vi "Test Task Rows.vi"(8 "error in":errorcluster, 10 "Work Folder":path, 11 "Test Data Folder":path) -> (0 "error out":errorcluster, 2 "Report":string, 3 "Passed":bool)   [LabVIEW 2026]
doc: "Tests Project Task Rows.vi and Apply Task Rows.vi on a copy of the schema-v2 sample data. Every check after a write reads the data back from disk with a fresh Initialize Stores.vi (Test - Read Task Rows.vi). The Meetings case and the unknown-ID case each run on their own copy. Checks: Client Website lists Design, Development and Testing in Sort Order with Testing inactive; Testing set active and Meetings (TimeTracker) set inactive survive re-reading; a new name (given with spaces, then repeated with Active FALSE) is added once and stays active; empty and blank names are ignored; tasks not in the rows keep their IDs and Active; an unknown Project ID gives error 5102 and leaves Tasks.ini as the sample it was copied from.\n\nInputs: Test Data Folder; Work Folder; error in. Outputs: Passed; Report; error out.\n\nGenerated by: Claude"
uses:
  UI Support/Task Edit Row.ctl
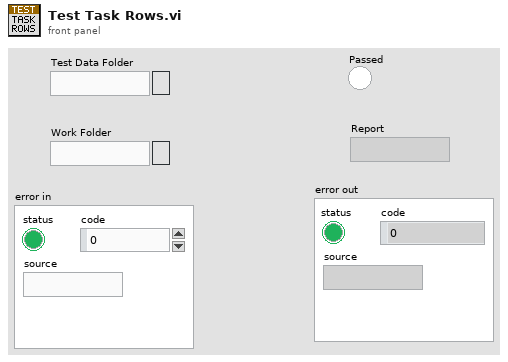
[diagram p1: front panel]
types:
  T1 = typedef "Task Edit Row.ctl" = cluster{"Task Name":string, "Active":bool}
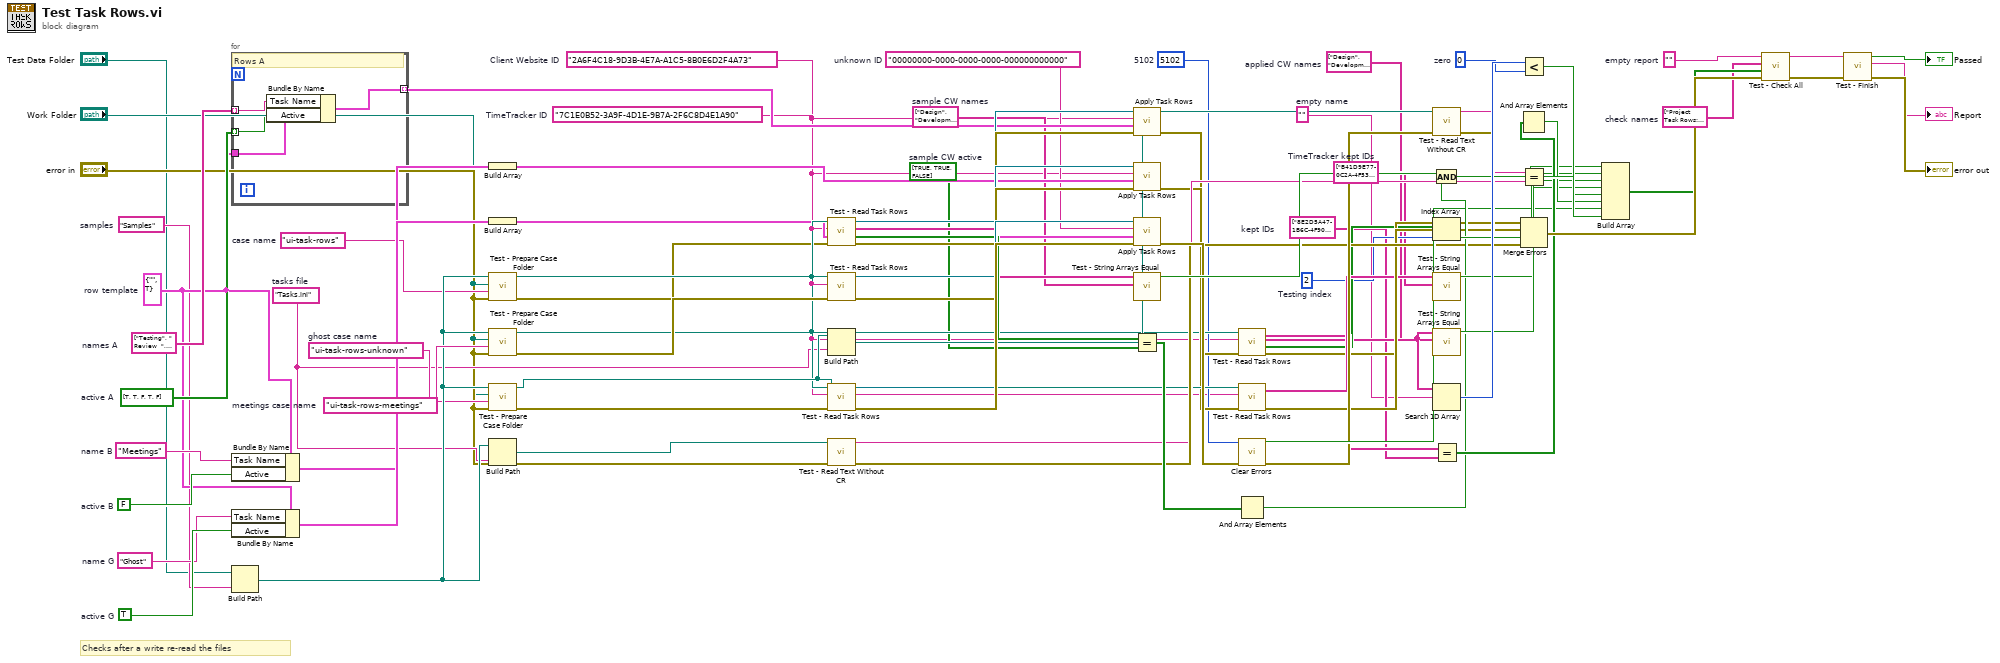
[diagram p0: block diagram]
diagram:
  w55 = "ui-task-rows-meetings"  # meetings case name
  w32 = "ui-task-rows-unknown"  # ghost case name
  w31 = 2  # Testing index
  w30 = string[] ["8E2D5A47-1B6C-4F90-8D3A-7C4B0E9F2A16", "14B9E6D3-A07C-4D52-9F18-3E6A5C2B8D70"]  # kept IDs
  w29 = string[] ["B41D9E77-0C2A-4F53-8E16-5A9D3C7B2E04", "5D8A2C90-7E14-4A6B-B3F9-0C6E1A4D7B25"]  # TimeTracker kept IDs
  w27 = string[] ["Project Task Rows: Client Website gives Design/Development/Testing in Sort Order with Testing inactive", "Apply Task Rows: Testing set active survives re-reading", "Apply Task Rows: Meetings set inactive survives re-reading", "Apply Task Rows: a new name is added once and a repeat in the rows is skipped", "Apply Task Rows: empty and blank names are ignored", "Apply Task Rows: tasks not in the rows keep their IDs and Active", "Apply Task Rows: unknown Project ID gives error 5102", "Apply Task Rows: unknown Project ID leaves Tasks.ini unchanged"]  # check names
  w26 = 5102  # 5102
  w25 = 0  # zero
  w24 = ""  # empty name
  w23 = string[] ["Design", "Development", "Testing", "Review"]  # applied CW names
  w22 = bool[] [TRUE, TRUE, FALSE]  # sample CW active
  w21 = string[] ["Design", "Development", "Testing"]  # sample CW names
  w20 = TRUE  # active G
  w19 = "Ghost"  # name G
  w18 = FALSE  # active B
  w17 = "Meetings"  # name B
  w16 = bool[] [TRUE, TRUE, FALSE, TRUE, FALSE]  # active A
  w15 = string[] ["Testing", "  Review  ", "Review", "", "   "]  # names A
  w14 = T1 {"Task Name"="", "Active"=TRUE}  # row template
  w13 = "00000000-0000-0000-0000-000000000000"  # unknown ID
  w12 = "7C1E0B52-3A9F-4D1E-9B7A-2F6C8D4E1A90"  # TimeTracker ID
  w11 = "2A6F4C18-9D3B-4E7A-A1C5-8B0E6D2F4A73"  # Client Website ID
  w10 = ""  # empty report
  w9 = "Tasks.ini"  # tasks file
  w8 = "ui-task-rows"  # case name
  w7 = "Samples"  # samples
  # "Checks after a write re-read the files"
  n1 = for {
    tunnel: w15 -> [w85] mode=indexing
    tunnel: w16 -> [w86] mode=indexing
    tunnel: w14 -> [w87]
    tunnel: [w88] -> w28 mode=indexing
    # "Rows A"
    n2 = Bundle By Name(cluster=w87, "Task Name"=w85, "Active"=w86) -> (w88:T1)
  }
  n3 = Bundle By Name(cluster=w14, "Task Name"=w17, "Active"=w18) -> (w33:T1)
  n4 = Bundle By Name(cluster=w14, "Task Name"=w19, "Active"=w20) -> (w35:T1)
  n5 = Build Path(base path="Test Data Folder", name or relative path=w7) -> (appended path=w37:path)
  n6 = Build Array(w33) -> (w34:T1[])
  n7 = Build Array(w35) -> (w36:T1[])
  n8 = call "Test - Prepare Case Folder.vi"("error in (no error)"="error in", "Case Name"=w8, "Work Folder"="Work Folder", "Source Folder"=w37) -> ("error out"=w38:errorcluster, "Case Folder"=w39:path)  [unwired: 6 in]
  n9 = call "Test - Prepare Case Folder.vi"("error in (no error)"="error in", "Case Name"=w55, "Work Folder"="Work Folder", "Source Folder"=w37) -> ("error out"=w56:errorcluster, "Case Folder"=w54:path)  [unwired: 6 in]
  n10 = call "Test - Prepare Case Folder.vi"("error in (no error)"="error in", "Case Name"=w32, "Work Folder"="Work Folder", "Source Folder"=w37) -> ("error out"=w57:errorcluster, "Case Folder"=w58:path)  [unwired: 6 in]
  n11 = Build Path(base path=w37, name or relative path=w9) -> (appended path=w60:path)
  n12 = call "Test - Read Task Rows.vi"("error in"=w38, "Project ID"=w11, "Data Folder"=w39) -> ("error out"=w43:errorcluster, "Active"=w42:bool[], "Task Names"=w41:string[], "Project Store out"=w40:refnum<class "Project Store.lvclass">)  [unwired: 4 in, 1 out]
  n13 = call "Test - Read Task Rows.vi"("error in"=w56, "Project ID"=w12, "Data Folder"=w54) -> ("error out"=w47:errorcluster, "Project Store out"=w46:refnum<class "Project Store.lvclass">)  [unwired: 4 in, 3 out]
  n14 = Build Path(base path=w58, name or relative path=w9) -> (appended path=w59:path)
  n15 = call "Test - Read Task Rows.vi"("error in"=w57, "Project ID"=w11, "Data Folder"=w58) -> ("error out"=w62:errorcluster, "Project Store out"=w61:refnum<class "Project Store.lvclass">)  [unwired: 4 in, 3 out]
  n16 = call "Test - Read Text Without CR.vi"("error in (no error)"="error in", "File"=w60) -> ("error out"=w64:errorcluster, "Text"=w63:string)  [unwired: 8 in]
  n17 = call "Apply Task Rows.vi"("error in"=w43, "Task Rows"=w28, "Project ID"=w11, "Project Store in"=w40) -> ("error out"=w44:errorcluster)  [unwired: 6 in, 1 out]
  n18 = call "Apply Task Rows.vi"("error in"=w47, "Task Rows"=w34, "Project ID"=w12, "Project Store in"=w46) -> ("error out"=w45:errorcluster)  [unwired: 6 in, 1 out]
  n19 = call "Apply Task Rows.vi"("error in"=w62, "Task Rows"=w36, "Project ID"=w13, "Project Store in"=w61) -> ("error out"=w65:errorcluster)  [unwired: 6 in, 1 out]
  n20 = call "Test - String Arrays Equal.vi"("Expected"=w21, "Actual"=w41) -> ("Equal?"=w70:bool)  [unwired: 8 in, 1 out]
  n21 = Equal?(x=w42, y=w22) -> (x = y?=w71:bool[])
  n22 = call "Test - Read Task Rows.vi"("error in"=w44, "Project ID"=w11, "Data Folder"=w39) -> ("error out"=w51:errorcluster, "Active"=w49:bool[], "Task Names"=w48:string[], "Active Task IDs"=w50:string[])  [unwired: 4 in, 1 out]
  n23 = call "Test - Read Task Rows.vi"("error in"=w45, "Project ID"=w12, "Data Folder"=w54) -> ("error out"=w53:errorcluster, "Active Task IDs"=w52:string[])  [unwired: 4 in, 3 out]
  n24 = call <vilib>:"Clear Errors.vi"("error in (no error)"=w65, "specific error code to clear (0: all)"=w26) -> ("error out"=w66:errorcluster, "specific error cleared?"=w67:bool)  [unwired: 4 in]
  n25 = And Array Elements(Boolean array=w71) -> (logical AND=w72:bool)
  n26 = call "Test - Read Text Without CR.vi"("error in (no error)"=w66, "File"=w59) -> ("error out"=w69:errorcluster, "Text"=w68:string)  [unwired: 8 in]
  n27 = And(x=w70, y=w72) -> (x .and. y?=w73:bool)
  n28 = Index Array(array=w49, index=w31) -> (element=w74:bool)
  n29 = call "Test - String Arrays Equal.vi"("Expected"=w29, "Actual"=w52) -> ("Equal?"=w75:bool)  [unwired: 8 in, 1 out]
  n30 = call "Test - String Arrays Equal.vi"("Expected"=w23, "Actual"=w48) -> ("Equal?"=w76:bool)  [unwired: 8 in, 1 out]
  n31 = Search 1D Array(1D array=w48, element=w24) -> (index of element=w77:i32)  [unwired: 1 in]
  n32 = Equal?(x=w50, y=w30) -> (x = y?=w79:bool[])
  n33 = Less?(x=w77, y=w25) -> (x < y?=w78:bool)
  n34 = And Array Elements(Boolean array=w79) -> (logical AND=w80:bool)
  n35 = Equal?(x=w68, y=w63) -> (x = y?=w81:bool)
  n36 = Merge Errors(w51, w53, w69, w64) -> (w83:errorcluster)
  n37 = Build Array(w73, w74, w75, w76, w78, w80, w67, w81) -> (w82:bool[])
  n38 = call "Test - Check All.vi"("Conditions"=w82, "Check Names"=w27, "Report in"=w10) -> ("Report out"=w84:string)  [unwired: 7 in, 1 out]
  n39 = call "Test - Finish.vi"("error in (no error)"=w83, "Report"=w84) -> ("error out"=→"error out":errorcluster, "Report out"=→"Report":string, "Passed"=→"Passed":bool)  [unwired: 7 in]
